vi "getBBsMasks.vi"(8 "error in (no error)":errorcluster, 9 "maskCounts":i32[](array[numeric]), 10 "bbCounts":i32[](array[numeric]), 11 "dl in":refnum<class "dl.lvclass">) -> (0 "error out":errorcluster, 2 "BatchResults":T1[](array[typedef]), 3 "dl out":refnum<class "dl.lvclass">)   [LabVIEW 2025, in "dl.lvlib" / "dl.lvclass"]
uses:
  dl.lvclass
  def/ImageResult.ctl
  detect.ctl
  def/Mask.ctl
  def/Polygon.ctl
  LVPointInt.ctl
  dl.lvclass/dl.ctl
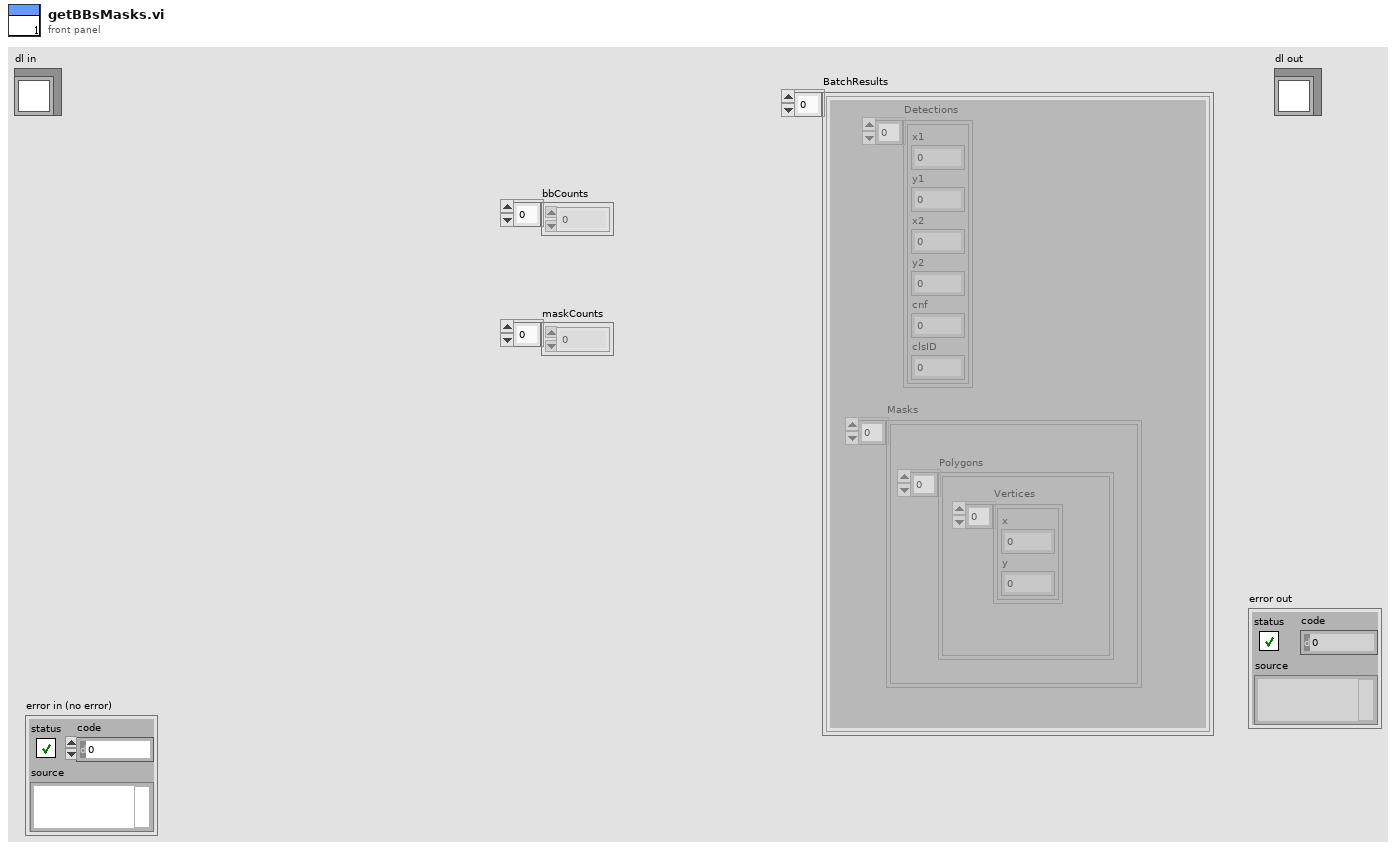
[diagram p1: front panel]
types:
  T1 = typedef "dl.lvlib/dl.lvclass/ImageResult.ctl" = cluster{"Detections":T2[], "Masks":T3[]}
  T2 = typedef "dl.lvlib/dl.lvclass/detect.ctl" = cluster{"x1":sgl, "y1":sgl, "x2":sgl, "y2":sgl, "cnf":sgl, "clsID":i32}
  T3 = typedef "dl.lvlib/dl.lvclass/Mask.ctl" = cluster{"Polygons":T4[]}
  T4 = typedef "dl.lvlib/dl.lvclass/Polygon.ctl" = cluster{"Vertices":T5[]}
  T5 = typedef "dl.lvlib/dl.lvclass/LVPointInt.ctl" = cluster{"x":i32, "y":i32}
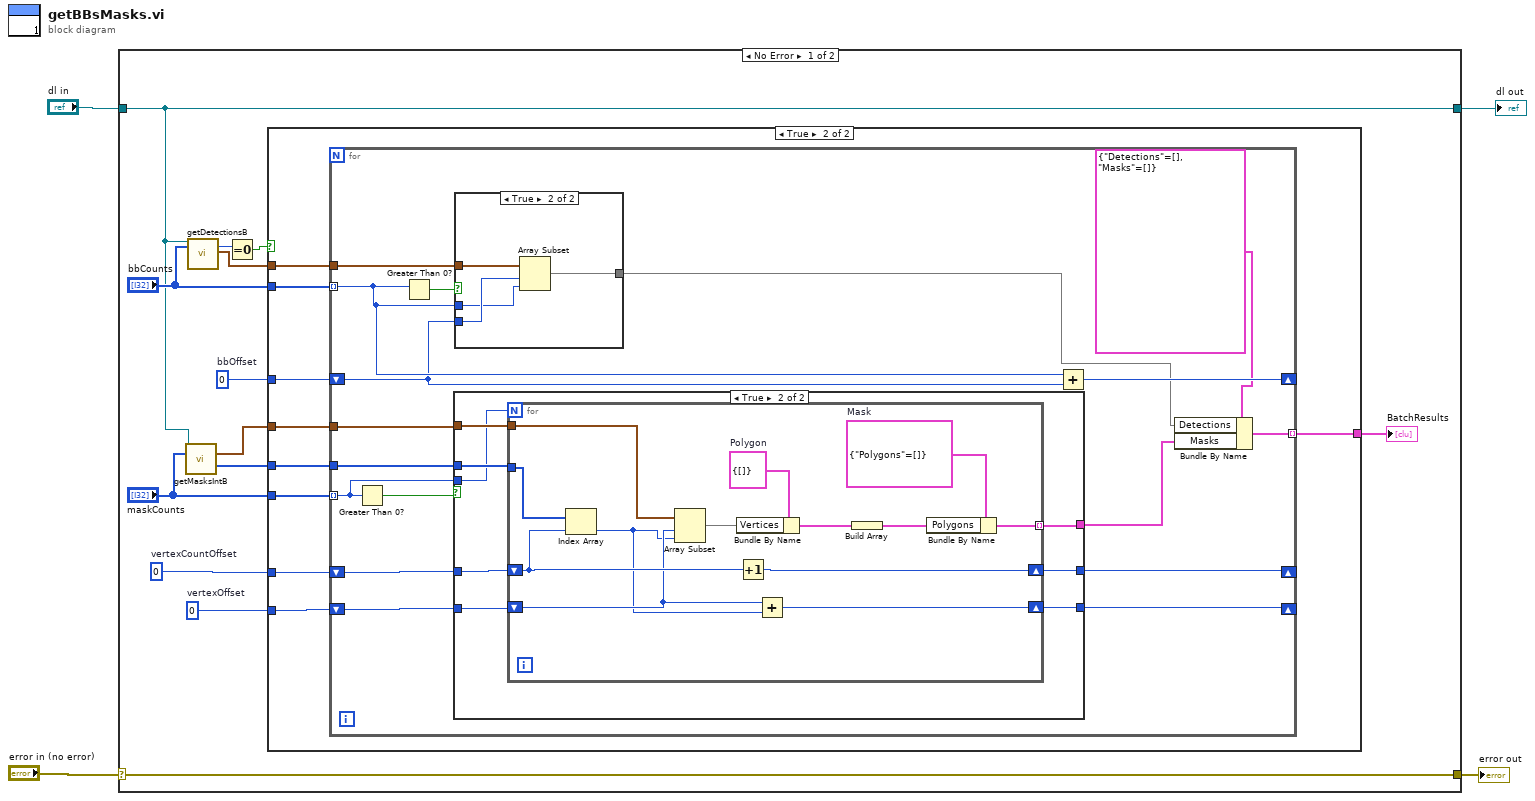
[diagram p0: block diagram]
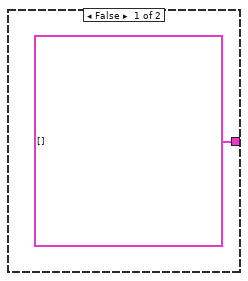
[diagram p2: hidden frame]
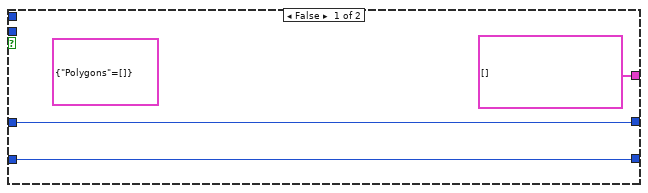
[diagram p3: hidden frame]
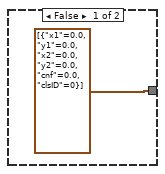
[diagram p4: hidden frame]
diagram:
  n1 = case shown="No Error" "error in (no error)" {
    selector: "error in (no error)" -> [w17 w75]
    tunnel: [w17 w75] -> w3
    tunnel: [w9 w74] -> w1
    tunnel: "dl in" -> [w9 w74]
    frame No Error {
      w14 = 0  # vertexOffset
      w15 = 0  # vertexCountOffset
      w16 = 0  # bbOffset
      n2 = call-dynamic "getMasksIntB.vi"("dl in"=w9, "maskCounts"="maskCounts") -> ("Vertices"=w6:T5[], "verticesPerPolygons"=w7:i32[])  [unwired: 9 in, 3 out]
      n3 = call-dynamic "getDetectionsB.vi"("dl in"=w9, "bbCounts"="bbCounts") -> ("succBB"=w12:i32, "detectionsBuffer"=w10:T2[])  [unwired: 12 in, 4 out]
      n4 = Equal To 0?(x=w12) -> (x = 0?=w11:bool)
      n5 = case shown="True" w11 {
        tunnel: w16 -> [_ w27]
        tunnel: w15 -> [_ w26]
        tunnel: w14 -> [_ w25]
        tunnel: "maskCounts" -> [_ w20]
        tunnel: "bbCounts" -> [_ w24]
        tunnel: w10 -> [_ w23]
        tunnel: w7 -> [_ w22]
        tunnel: w6 -> [_ w21]
        tunnel: [T1[] [] w19] -> w5
        frame False {
        }
        frame True {
          n6 = for {
            tunnel: w24 -> [w42] mode=indexing
            shift-right: [w40] -> _
            shift-left: w27 -> [w41]
            shift-right: [w33] -> _
            shift-left: w26 -> [w38]
            shift-right: [w32] -> _
            shift-left: w25 -> [w37]
            tunnel: w20 -> [w34] mode=indexing
            tunnel: w23 -> [w43]
            tunnel: w22 -> [w36]
            tunnel: w21 -> [w35]
            tunnel: [w28] -> w19 mode=indexing
            n7 = Greater Than 0?(x=w34) -> (x > 0?=w39:bool)
            n8 = Greater Than 0?(x=w42) -> (x > 0?=w44:bool)
            n9 = case shown="True" w39 {
              tunnel: [T3[] [] w50] -> w29
              tunnel: w38 -> [w46 w55]
              tunnel: w37 -> [w45 w54]
              tunnel: w36 -> [_ w53]
              tunnel: w35 -> [_ w52]
              tunnel: w34 -> [_ w51]
              tunnel: [w46 w49] -> w33
              tunnel: [w45 w48] -> w32
              frame False {
                (unwired) T3 {"Polygons"=[]} ("Mask")
              }
              frame True {
                n10 = for {
                  N: w51 -> [_]
                  shift-right: [w59] -> w49
                  shift-left: w55 -> [w60]
                  shift-right: [w56] -> w48
                  shift-left: w54 -> [w58]
                  tunnel: w53 -> [w68]
                  tunnel: w52 -> [w67]
                  tunnel: [w61] -> w50 mode=indexing
                  w64 = T3 {"Polygons"=[]}  # Mask
                  w66 = T4 {"Vertices"=[]}  # Polygon
                  n11 = Index Array(array=w68, index=w60) -> (element=w57:i32)
                  n12 = Array Subset(array=w67, index=w58, length=w57) -> (w65:T5[])
                  n13 = Bundle By Name(cluster=w66, "Vertices"=w65) -> (w63:T4)
                  n14 = Increment(x=w60) -> (x+1=w59:i32)
                  n15 = Add(x=w58, y=w57) -> (x+y=w56:i32)
                  n16 = Build Array(w63) -> (w62:T4[])
                  n17 = Bundle By Name(cluster=w64, "Polygons"=w62) -> (w61:T3)
                }
              }
            }
            n18 = case shown="True" w44 {
              tunnel: w43 -> [_ w73]
              tunnel: w41 -> [_ w72]
              tunnel: w42 -> [_ w71]
              tunnel: [T2[] [{"x1"=0.0, "y1"=0.0, "x2"=0.0, "y2"=0.0, "cnf"=0.0, "clsID"=0}] w70] -> w30
              frame False {
              }
              frame True {
                n19 = Array Subset(array=w73, index=w72, length=w71) -> (w70:T2[])
              }
            }
            n20 = Add(x=w42, y=w41) -> (x+y=w40:i32)
            n21 = Bundle By Name(cluster=T1 {"Detections"=[], "Masks"=[]} ("ImageResult"), "Detections"=w30, "Masks"=w29) -> (w28:T1)
          }
        }
      }
      "BatchResults" <- w5
    }
    frame Error {
    }
  }
  "error out" <- w3
  "dl out" <- w1
